vi "main.vi"() -> ()   [LabVIEW 2022 SP3]
uses:
  <vilib>/Waveform/WDTOps.llb/WDT Append Waveforms DBL.vi
  global_variant.vi
  <vilib>/Waveform/WDTFileIO.llb/Write Waveforms to File (1D).vi
  <vilib>/measure/NI_MABase.lvlib
panel:
  in  "locking":bool
  out "是否采集结束":bool
  out "是否采集":bool
  in  "数据回放":bool
  in  "数据记录":bool
  in  "采集数据":bool
  in  "电压基准（V/div）":dbl(knob)=2.0 step=1.0 scale=1.0..4.0
  in  "时间基准（ms/div）":dbl(knob)=25.0 step=5.0 scale=5.0..25.0
  in  "CH2":enum16{"三角波", "方波", "正弦波", "锯齿波"}(ring)=enum."方波"
  in  "标准差(V)":dbl(knob)=0.025700497905212782 scale=0.0..0.2
  in  "直流分量(V)":dbl(knob) scale=-1.0..1.0
  out "通道二灯":bool
  in  "通道2开关":bool=TRUE
  in  "幅值(V)":dbl(knob)=3.0773807796628723 scale=0.0..10.0
  in  "频率(Hz)":dbl(knob)=23.226445379934056 scale=0.0..200.0
  in  "直流分量(V)":dbl(knob) scale=-1.0..1.0
  in  "标准差(V)":dbl(knob)=0.09289109030690795 scale=0.0..0.2
  in  "CH1":enum16{"三角波", "方波", "正弦波", "锯齿波"}(ring)
  in  "幅值(V)":dbl(knob)=3.7121438310672197 scale=0.0..10.0
  in  "频率(Hz)":dbl(knob)=29.199821580820895 scale=0.0..200.0
  in  "通道1开关":bool=TRUE
  out "通道一灯":bool
  in  "退出系统":bool
  out "波形":waveform(dbl)[](graph)
  # "双通道数据采集处理系统"
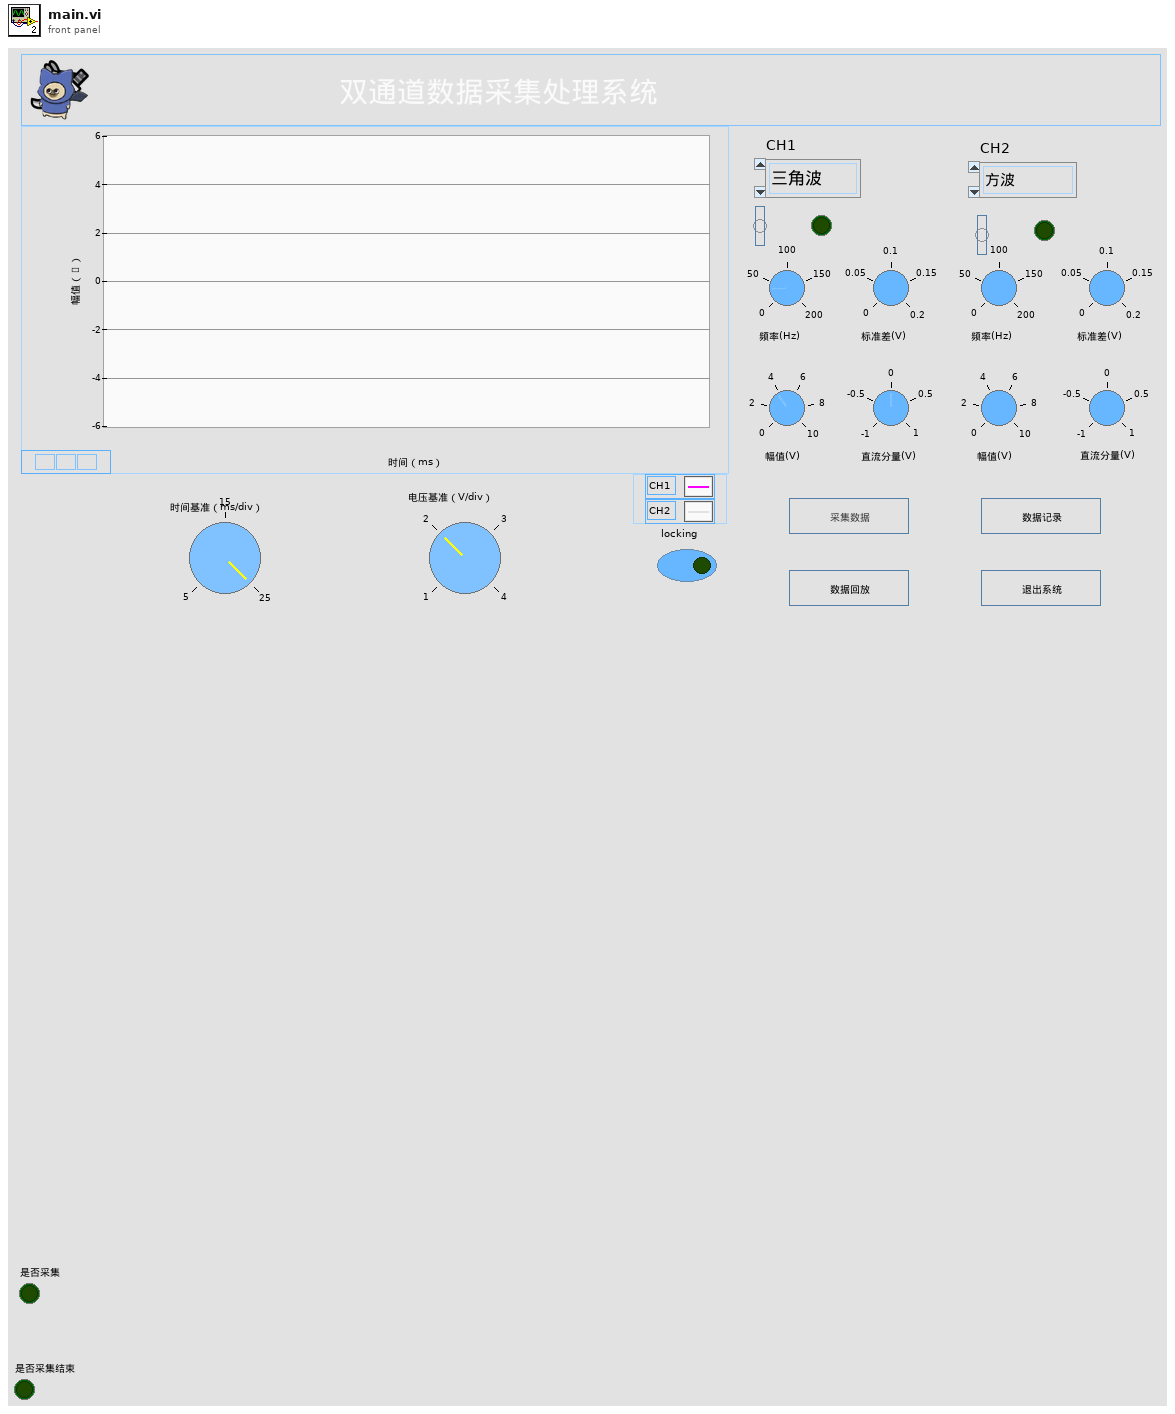
[diagram p1: front panel]
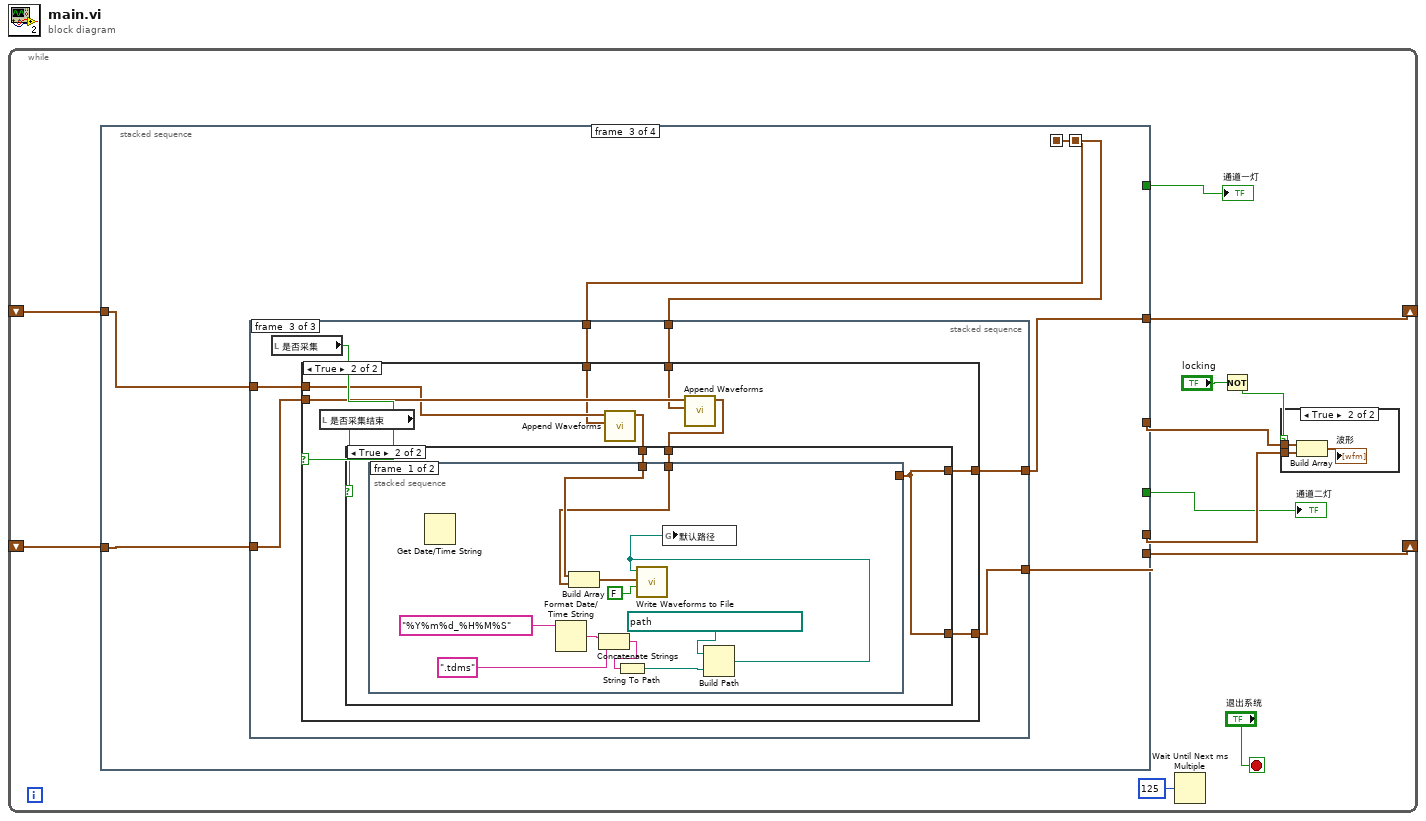
[diagram p0: block diagram]
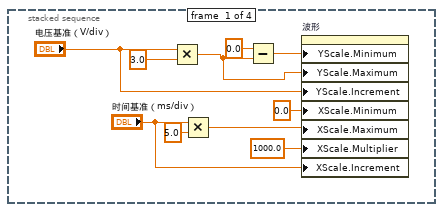
[diagram p3: hidden frame]
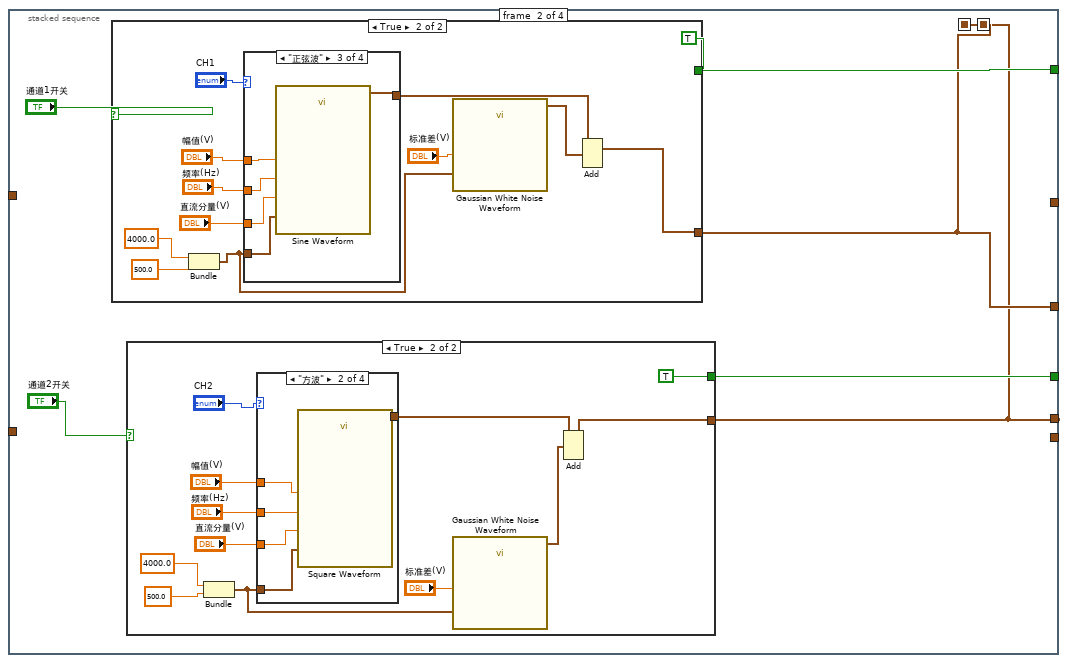
[diagram p4: hidden frame]
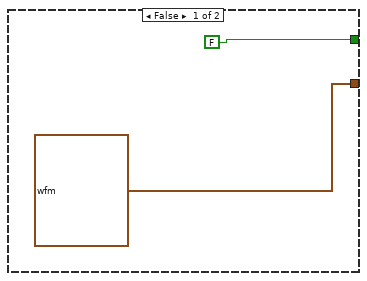
[diagram p5: hidden frame]
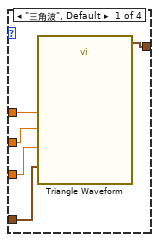
[diagram p6: hidden frame]
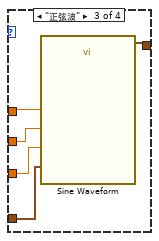
[diagram p7: hidden frame]
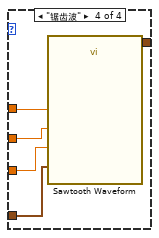
[diagram p8: hidden frame]
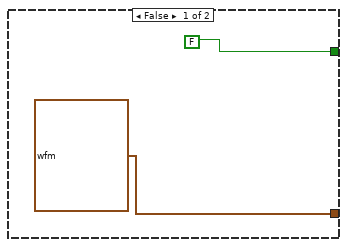
[diagram p9: hidden frame]
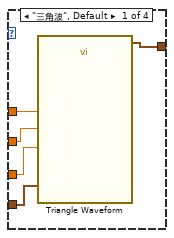
[diagram p10: hidden frame]
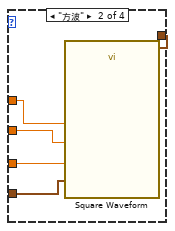
[diagram p11: hidden frame]
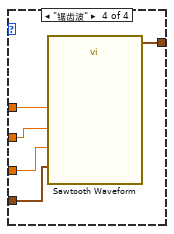
[diagram p12: hidden frame]
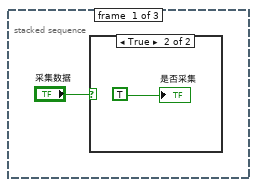
[diagram p13: hidden frame]
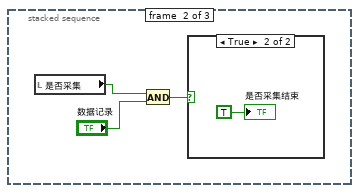
[diagram p15: hidden frame]
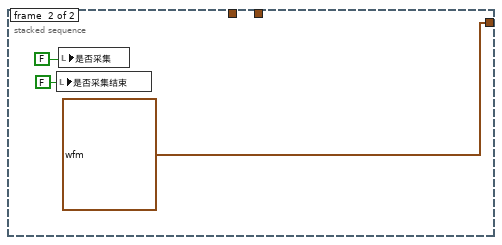
[diagram p19: hidden frame]
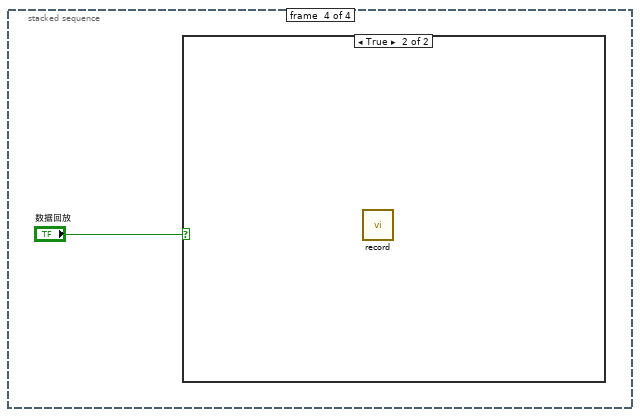
[diagram p20: hidden frame]
diagram:
  n1 = while {
    shift-right: [w1] -> _
    shift-left: _ -> [w8]
    shift-right: [w2] -> _
    shift-left: _ -> [w7]
    stop <- "退出系统" stop-if-true
    n2 = stacked-sequence {
      seq-local: [_ w26 _ _] -> [_ _ w105 _]
      seq-local: [_ w27 _ _] -> [_ _ w101 _]
      tunnel: [_ w27 _ _] -> w12
      tunnel: [_ w26 _ _] -> w11
      tunnel: [_ w29 _ _] -> w10
      tunnel: [_ w28 _ _] -> w9
      tunnel: w8 -> [_ _ w102 _]
      tunnel: w7 -> [_ _ w100 _]
      tunnel: [_ _ w104 _] -> w2
      tunnel: [_ _ w103 _] -> w1
      frame #0 {
        n3 = Multiply(x="电压基准（V/div）", y=3.0) -> (x*y=w18:dbl)
        n4 = Multiply(x="时间基准（ms/div）", y=5.0) -> (x*y=w20:dbl)
        n5 = Subtract(x=0.0, y=w18) -> (x-y=w17:dbl)
        n6 = property on="波形" class="WFGraph (strict)"("YScale.Minimum"=w17, "YScale.Maximum"=w18, "YScale.Increment"="电压基准（V/div）", "XScale.Minimum"=0.0, "XScale.Maximum"=w20, "XScale.Multiplier"=1000.0, "XScale.Increment"="时间基准（ms/div）") -> ()  [unwired: 2 in, 2 out]
      }
      frame #1 {
        n7 = case shown="True" "通道1开关" {
          tunnel: [FALSE TRUE] -> w28
          tunnel: [waveform(dbl) {"t0"=timestamp(0 s since 1904-01-01), "dt"=1.0, "Y"=[]} ("Waveform") w68] -> w27
          frame False {
          }
          frame True {
            n8 = Bundle(4000.0, 500.0) -> (w69:cluster{dbl, dbl})  [unwired: 1 in]
            n9 = case shown="\"正弦波\"" "CH1" {
              tunnel: "幅值(V)" -> [w84 w89 w94 w99]
              tunnel: "频率(Hz)" -> [w83 w88 w93 w98]
              tunnel: [w82 w87 w92 w97] -> w73
              tunnel: "直流分量(V)" -> [w81 w86 w91 w96]
              tunnel: w69 -> [w80 w85 w90 w95]
              frame "三角波", Default {
                n10 = call <vilib>:"Triangle Waveform.vi"("offset"=w81, "sampling info"=w80, "amplitude"=w84, "frequency"=w83) -> ("signal out"=w82:waveform(dbl))  [unwired: 6 in, 1 out]
              }
              frame "方波" {
                n11 = call <vilib>:"Square Waveform.vi"("offset"=w86, "sampling info"=w85, "amplitude"=w89, "frequency"=w88) -> ("signal out"=w87:waveform(dbl))  [unwired: 6 in, 1 out]
              }
              frame "正弦波" {
                n12 = call <vilib>:"Sine Waveform.vi"("offset"=w91, "sampling info"=w90, "amplitude"=w94, "frequency"=w93) -> ("signal out"=w92:waveform(dbl))  [unwired: 6 in, 1 out]
              }
              frame "锯齿波" {
                n13 = call <vilib>:"Sawtooth Waveform.vi"("offset"=w96, "sampling info"=w95, "amplitude"=w99, "frequency"=w98) -> ("signal out"=w97:waveform(dbl))  [unwired: 6 in, 1 out]
              }
            }
            n14 = call <vilib>:"Gaussian White Noise Waveform.vi"("sampling info"=w69, "standard deviation"="标准差(V)") -> ("signal out"=w74:waveform(dbl))  [unwired: 8 in, 1 out]
            n15 = Add(1:w74, 2:w73) -> (0:w68:waveform(dbl))  [unwired: 1 in, 1 out]
          }
        }
        n16 = case shown="True" "通道2开关" {
          tunnel: [FALSE TRUE] -> w29
          tunnel: [waveform(dbl) {"t0"=timestamp(0 s since 1904-01-01), "dt"=1.0, "Y"=[]} ("Waveform") w34] -> w26
          frame False {
          }
          frame True {
            n17 = Bundle(4000.0, 500.0) -> (w35:cluster{dbl, dbl})  [unwired: 1 in]
            n18 = case shown="\"方波\"" "CH2" {
              tunnel: [w50 w55 w60 w65] -> w43
              tunnel: "直流分量(V)" -> [w49 w52 w59 w64]
              tunnel: "频率(Hz)" -> [w48 w53 w58 w63]
              tunnel: "幅值(V)" -> [w47 w54 w57 w62]
              tunnel: w35 -> [w46 w51 w56 w61]
              frame "三角波", Default {
                n19 = call <vilib>:"Triangle Waveform.vi"("offset"=w49, "sampling info"=w46, "amplitude"=w47, "frequency"=w48) -> ("signal out"=w50:waveform(dbl))  [unwired: 6 in, 1 out]
              }
              frame "方波" {
                n20 = call <vilib>:"Square Waveform.vi"("offset"=w52, "sampling info"=w51, "amplitude"=w54, "frequency"=w53) -> ("signal out"=w55:waveform(dbl))  [unwired: 6 in, 1 out]
              }
              frame "正弦波" {
                n21 = call <vilib>:"Sine Waveform.vi"("offset"=w59, "sampling info"=w56, "amplitude"=w57, "frequency"=w58) -> ("signal out"=w60:waveform(dbl))  [unwired: 6 in, 1 out]
              }
              frame "锯齿波" {
                n22 = call <vilib>:"Sawtooth Waveform.vi"("offset"=w64, "sampling info"=w61, "amplitude"=w62, "frequency"=w63) -> ("signal out"=w65:waveform(dbl))  [unwired: 6 in, 1 out]
              }
            }
            n23 = call <vilib>:"Gaussian White Noise Waveform.vi"("sampling info"=w35, "standard deviation"="标准差(V)") -> ("signal out"=w38:waveform(dbl))  [unwired: 8 in, 1 out]
            n24 = Add(1:w38, 2:w43) -> (0:w34:waveform(dbl))  [unwired: 1 in, 1 out]
          }
        }
      }
      frame #2 {
        n25 = stacked-sequence {
          tunnel: w105 -> [_ _ w117]
          tunnel: [_ _ w116] -> w104
          tunnel: [_ _ w115] -> w103
          tunnel: w102 -> [_ _ w114]
          tunnel: w101 -> [_ _ w113]
          tunnel: w100 -> [_ _ w112]
          frame #0 {
            n26 = case shown="True" "采集数据" {
              frame False {
              }
              frame True {
                "是否采集" <- TRUE
              }
            }
          }
          frame #1 {
            n27 = local read "是否采集"() -> (w109:bool)
            n28 = And(x=w109, y="数据记录") -> (x .and. y?=w108:bool)
            n29 = case shown="True" w108 {
              frame False {
              }
              frame True {
                "是否采集结束" <- TRUE
              }
            }
          }
          frame #2 {
            n30 = local read "是否采集"() -> (w118:bool)
            n31 = case shown="True" w118 {
              tunnel: w117 -> [w120 w123]
              tunnel: [w119 w128] -> w116
              tunnel: [w120 w127] -> w115
              tunnel: w114 -> [_ w124]
              tunnel: w113 -> [w119 w121]
              tunnel: w112 -> [_ w122]
              frame False {
              }
              frame True {
                n32 = local read "是否采集结束"() -> (w129:bool)
                n33 = call-poly <vilib>:"Append Waveforms.vi"("waveform B"=w121, "waveform A"=w122) -> ("waveform out"=w126:waveform(dbl))  [unwired: 8 in, 1 out]
                n34 = call-poly <vilib>:"Append Waveforms.vi"("waveform B"=w123, "waveform A"=w124) -> ("waveform out"=w125:waveform(dbl))  [unwired: 8 in, 1 out]
                n35 = case shown="True" w129 {
                  tunnel: w126 -> [w131 w133]
                  tunnel: w125 -> [w130 w132]
                  tunnel: [w131 w134] -> w128
                  tunnel: [w130 w134] -> w127
                  frame False {
                  }
                  frame True {
                    n36 = stacked-sequence {
                      tunnel: [_ waveform(dbl) {"t0"=timestamp(0 s since 1904-01-01), "dt"=1.0, "Y"=[]} ("Waveform")] -> w134
                      tunnel: w133 -> [w144 _]
                      tunnel: w132 -> [w143 _]
                      frame #0 {
                        n37 = Get Date/Time String() -> ()  [unwired: 3 in, 2 out]
                        n38 = Format Date/Time String(time format string (%c)="%Y%m%d_%H%M%S") -> (date/time string=w140:string)  [unwired: 2 in]
                        n39 = Build Array(w144, w143) -> (w142:waveform(dbl)[])
                        n40 = Concatenate Strings(w140, ".tdms" ("time format string (%c)")) -> (w138:string)
                        n41 = String To Path(string=w138) -> (path=w136:path)
                        n42 = Build Path(base path=path "D:/学校/LabView/DDS/saves" ("file path (dialog if empty)"), name or relative path=w136) -> (appended path=w135:path)
                        n43 = call-poly <vilib>:"Write Waveforms to File.vi"("append to file? (new file:F)"=FALSE, "waveform array"=w142, "file path (dialog if empty)"=w135) -> ()  [unwired: 7 in, 2 out]
                        n44 = global write "global_variant.vi" "默认路径"(w135) -> ()
                      }
                      frame #1 {
                        n45 = local write "是否采集结束"(FALSE) -> ()
                        n46 = local write "是否采集"(FALSE) -> ()
                      }
                    }
                  }
                }
              }
            }
          }
        }
      }
      frame #3 {
        n47 = case shown="True" "数据回放" {
          frame False {
          }
          frame True {
            n48 = call "record.vi"() -> ()  [unwired: 12 in]
          }
        }
      }
    }
    "通道二灯" <- w10
    "通道一灯" <- w9
    n49 = Wait Until Next ms Multiple(millisecond multiple=u32 125) -> ()  [unwired: 1 out]
    n50 = Not(x="locking") -> (.not. x?=w4:bool)
    n51 = case shown="True" w4 {
      tunnel: w12 -> [_ w14]
      tunnel: w11 -> [_ w13]
      frame False {
      }
      frame True {
        n52 = Build Array(w14, w13) -> (→"波形":waveform(dbl)[])
      }
    }
  }
